vi "XML - Create XML file.vi"(8 "error in (no error)":errorcluster, 10 "Consolidated_CD":refnum<class "NIVS_Consolidated_CDW_MetaDataObj.lvclass">, 11 "CD Wizard - Internal Data":T1) -> (0 "error out":errorcluster)   [LabVIEW 2020, in "NIVS_Consolidated_CDW_MetaDataObj.lvclass"]
doc: "Create the XML file and alter the content of the file, so that it fits for the generated custom device."
uses:
  NIVS_Consolidated_CDW_MetaDataObj.lvclass
  Internal data.ctl
  C:/Program Files/National Instruments/LabVIEW 2024/resource/dialog/NewProjectWizard/MetaDataObj/MetaDataObj.lvclass
  Create XML-file - States.ctl
  <resource>/dialog/NewProjectWizard/MetaDataObj/MetaDataObj.lvclass/MetaDataObj.ctl
  NIVS_Consolidated_CDW_MetaDataObj.lvclass/NIVS_Consolidated_CDW_MetaDataObj.ctl
  Template Classes/NIVS_CD Template/NIVS_CD Template.lvclass/NIVS_CD Template.ctl
  CD System Explorer lvlib.ctl
  Target Type.ctl
  Template Classes/NIVS_CD Template/Read Submenu.vi
  Template Classes/NIVS_CD Template/Read Parent Menu.vi
  Template Classes/NIVS_CD Template/Read Max Instances.vi
  <resource>/dialog/NewProjectWizard/MetaDataObj/Accessors/Read Project Root.vi
  <resource>/dialog/NewProjectWizard/MetaDataObj/Accessors/Read Project Name.vi
  Read CD Template.vi
  CD System Explorer lvlib.vi
  Template Classes/NIVS_CD Template/NIVS_CD Template.lvclass
  <vilib>/Utility/Data Type/NI_Data Type.lvlib
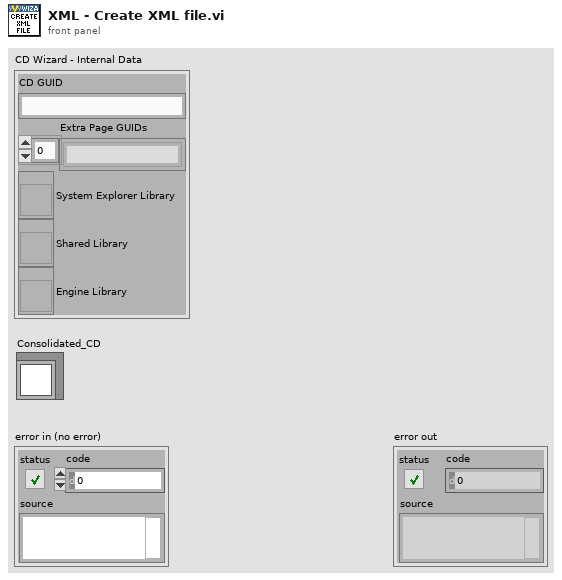
[diagram p1: front panel]
types:
  T1 = typedef "NIVS_Consolidated_CDW_MetaDataObj.lvclass/Internal data.ctl" = cluster{"CD GUID":string, "Extra Page GUIDs":string[], "System Explorer Library":refnum<vi>, "Shared Library":refnum<vi>, "Engine Library":refnum<vi>}
  T2 = typedef "NIVS_Consolidated_CDW_MetaDataObj.lvclass/Create XML-file - States.ctl" = enum16{"Read XML template file", "Change CD -MenuName-", "Change CD -Name-", "Change CD -Type-", "Change CD -Occurrences-", "Change CD -MainPageGUID-", "Change CD -InitVIPath-", "Change CD -WindowsCustomDeviceVIPath-", "Change CD -WindowsCustomDeviceVIRTPath-", "Change CD -Linuxx64CustomDeviceVIPath-", "Change CD -Linuxx64CustomDeviceVIRTPath-", "Change CD -MainPageVIPath-", "Change CD -ExtraPages-", "Change CD -ActionVIOnCompile-", "Change CD -ActionVIOnRecompile-", "Change CD -ExportConfigurationRTM-", "Write XML file content back"}
  T3 = typedef "NIVS_Consolidated_CDW_MetaDataObj.lvclass/CD System Explorer lvlib.ctl" = enum16{"LibraryFileName", "LibraryFolderName", "System Explorer.FolderName", "System Explorer.Dynamically Called.FolderName", "System Explorer.Dynamically Called.Extra Pages.FolderName", "System Explorer.Dynamically Called.Extra Pages.TemplatePathAndName", "System Explorer.Dynamically Called.Main Page.VIName", "System Explorer.Dynamically Called.Main Page.TemplatePathAndName", "System Explorer.Dynamically Called.Initialization VI.VIName", "System Explorer.Dynamically Called.Initialization VI.TemplatePathAndName", "System Explorer.SubVI.FolderName", "System Explorer.Types.FolderName", "System Explorer.ActionVIOnCompile.VIName", "System Explorer.ActionVIOnRecompile.VIName", "System Explorer.ExportConfigRTM.VIName", "System Explorer.PPL.ExportConfigRTM.VIName", "System Explorer.LoadHelpFile.VIName", "System Explorer.PPL.LoadHelpFile.VIName", "System Explorer.SetRTDriverVIsFilePaths.VIName", "System Explorer.ClearRTDriverVIs.VIName"}
  T4 = typedef "NIVS_Consolidated_CDW_MetaDataObj.lvclass/Target Type.ctl" = enum16{"Windows", "Linux x64"}
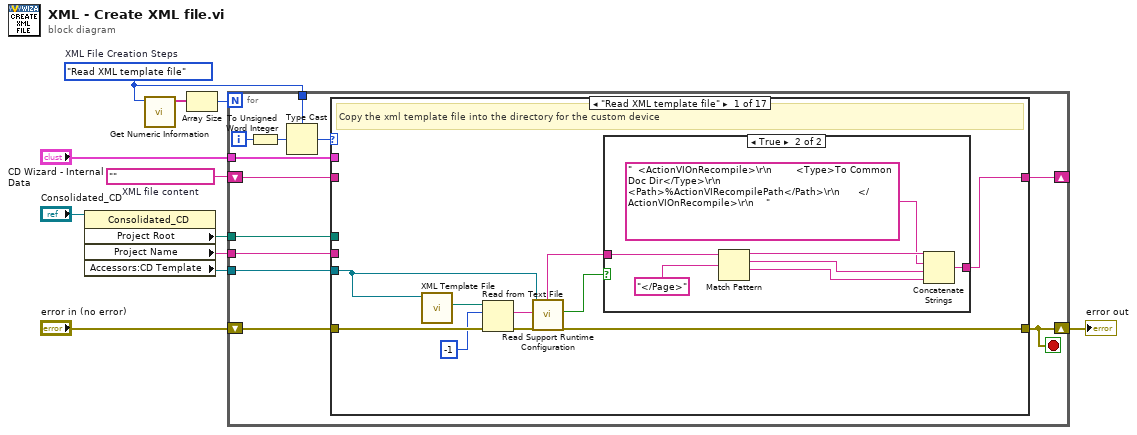
[diagram p0: block diagram]
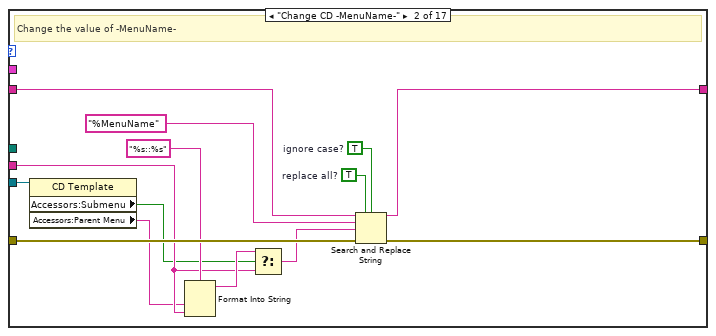
[diagram p3: hidden frame]
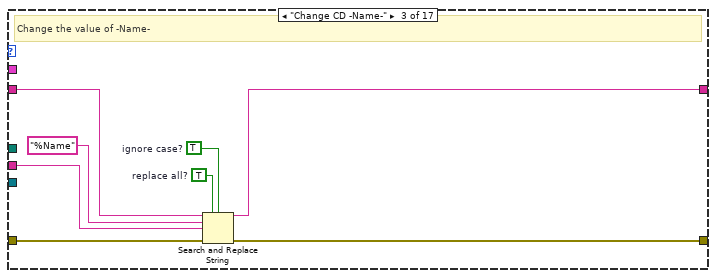
[diagram p4: hidden frame]
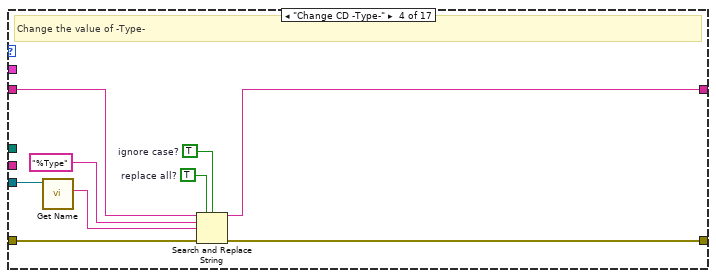
[diagram p5: hidden frame]
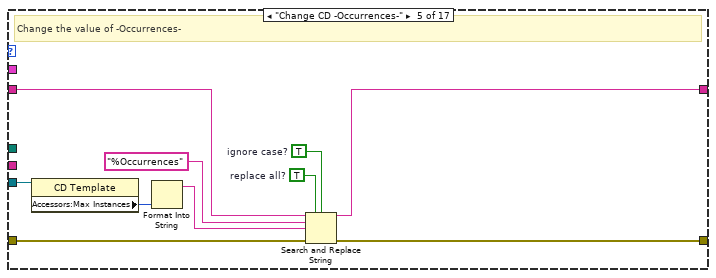
[diagram p6: hidden frame]
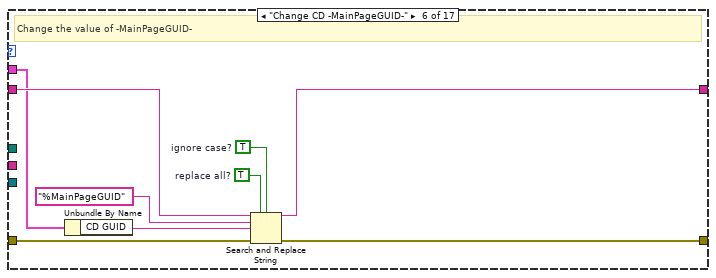
[diagram p7: hidden frame]
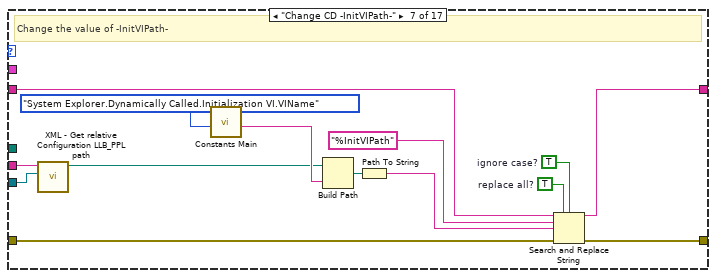
[diagram p8: hidden frame]
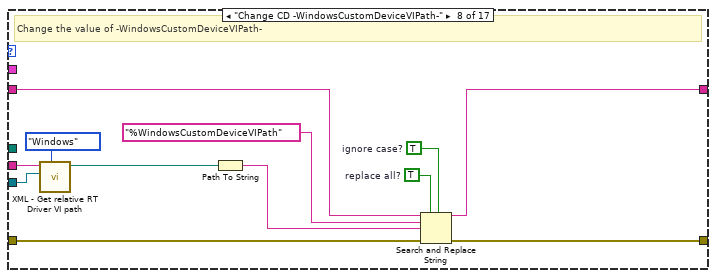
[diagram p9: hidden frame]
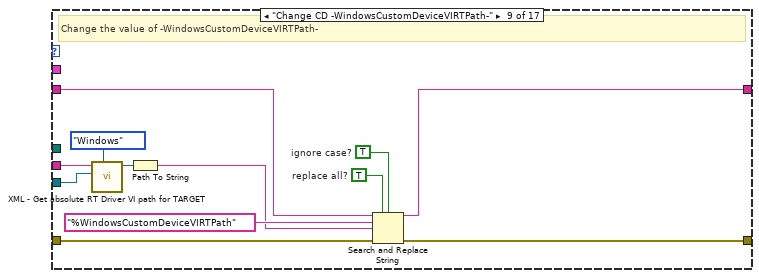
[diagram p10: hidden frame]
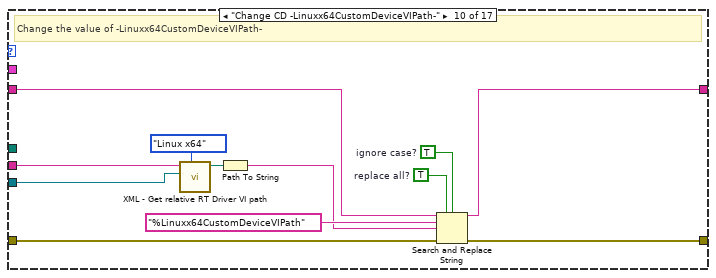
[diagram p11: hidden frame]
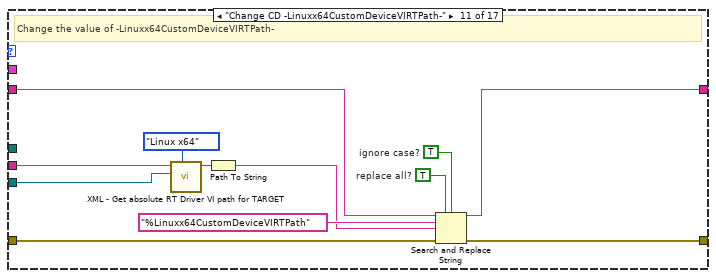
[diagram p12: hidden frame]
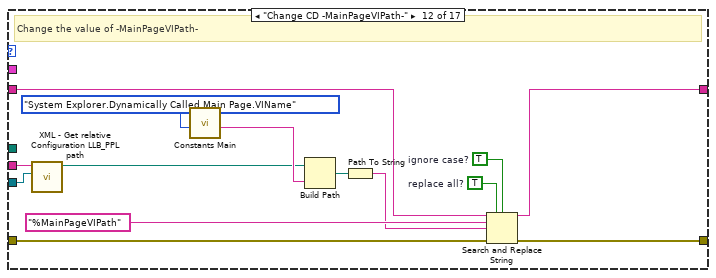
[diagram p13: hidden frame]
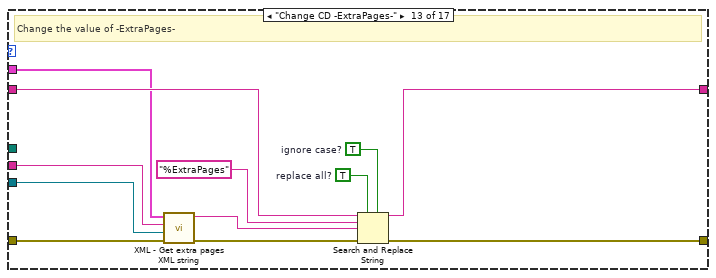
[diagram p14: hidden frame]
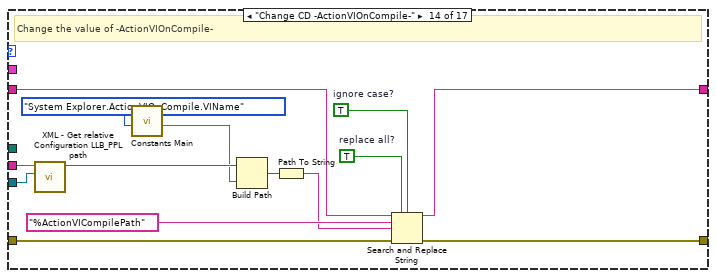
[diagram p15: hidden frame]
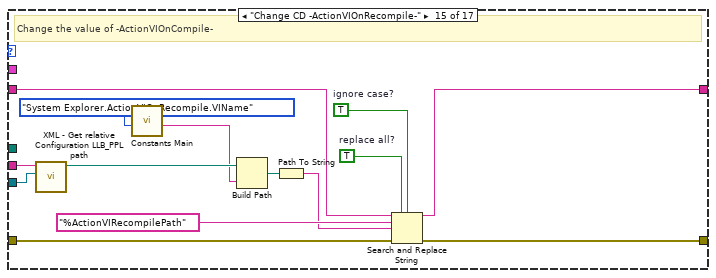
[diagram p16: hidden frame]
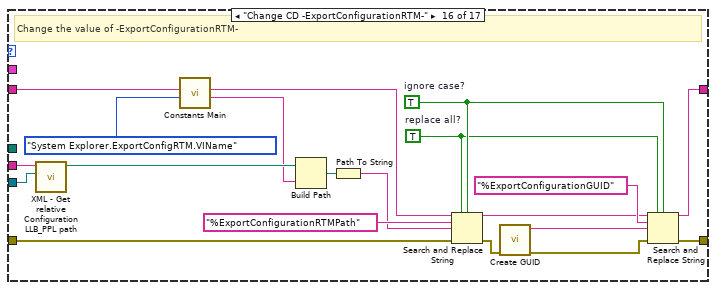
[diagram p17: hidden frame]
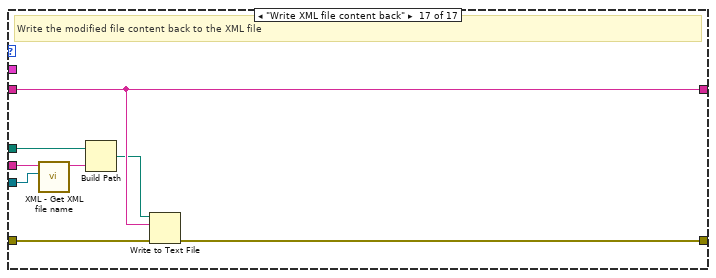
[diagram p18: hidden frame]
diagram:
  w2 = Create_XML-file_-_States."Read XML template file"  # XML File Creation Steps
  w10 = ""  # XML file content
  n1 = property class="Consolidated_CD"(reference="Consolidated_CD") -> ("Project Root"=w8:path, "Project Name"=w7:string, "Accessors:CD Template"=w6:refnum<class "NIVS_CD Template.lvclass">)  [unwired: 1 in, 2 out]
  n2 = call <vilib>:"Get Numeric Information.vi"("variant"=w2) -> ("enum names"=w3:string[])  [unwired: 7 in, 3 out]
  n3 = Array Size(array=w3) -> (size(s)=w4:i32)
  n4 = for {
    N: w4 -> [_]
    shift-right: [w18] -> w11
    shift-left: "error in (no error)" -> [w17]
    shift-right: [w22] -> _
    shift-left: w10 -> [w23]
    tunnel: w8 -> [w21]
    tunnel: w7 -> [w20]
    tunnel: w6 -> [w19]
    tunnel: w2 -> [w15]
    tunnel: "CD Wizard - Internal Data" -> [w12]
    i -> [w16]
    stop <- w18 stop-if-true
    # "While loop for State Machine"
    n5 = To Unsigned Word Integer(number=w16) -> (unsigned 16bit integer=w14:u16)
    n6 = Type Cast(type=w15, x=w14) -> (*(type *) &x=w13:T2)
    n7 = case shown="\"Read XML template file\"" w13 {
      tunnel: w17 -> [w32 w50 w58 w65 w72 w83 w93 w107 w119 w131 w143 w155 w169 w179 w193 w207 w230]
      tunnel: [w24 w51 w59 w68 w78 w87 w101 w115 w126 w138 w150 w163 w175 w189 w203 w210 w233] -> w18
      tunnel: w12 -> [_ _ _ _ _ w86 _ _ _ _ _ _ w173 _ _ _ _]
      tunnel: w23 -> [_ w53 w61 w70 w80 w89 w103 w112 w128 w140 w152 w165 w177 w191 w205 w224 w232]
      tunnel: [w28 w52 w60 w69 w79 w88 w102 w116 w127 w139 w151 w164 w176 w190 w204 w214 w232] -> w22
      tunnel: w21 -> [_ _ _ _ _ _ _ _ _ _ _ _ _ _ _ _ w229]
      tunnel: w20 -> [_ w44 w55 _ _ _ w92 w106 w118 w130 w142 w154 w168 w181 w195 w209 w228]
      tunnel: w19 -> [w27 w43 _ w64 w74 _ w91 w105 w117 w129 w141 w153 w167 w180 w194 w208 w227]
      frame "Read XML template file" {
        # "Copy the xml template file into the directory for the custom device"
        n8 = call-dynamic "XML Template File.vi"("CD Template"=w27) -> ("XML Template File"=w31:path)  [unwired: 10 in]
        n9 = Read from Text File(file (use dialog)=w31, count=-1, error in=w32) -> (text=w29:string, error out=w26:errorcluster)  [unwired: 1 in, 2 out]
        n10 = call "Read Support Runtime Configuration.vi"("error in"=w26, "NIVS_CD Template in"=w27) -> ("error out"=w24:errorcluster, "Support Runtime Configuration"=w25:bool)  [unwired: 7 in, 1 out]
        n11 = case shown="True" w25 {
          tunnel: w29 -> [w33 w37]
          tunnel: [w33 w36] -> w28
          frame False {
          }
          frame True {
            n12 = Match Pattern(string=w37, regular expression="</Page>" ("string")) -> (before substring=w40:string, match substring=w39:string, after substring=w34:string)  [unwired: 1 in, 1 out]
            n13 = Concatenate Strings(w40, "  <ActionVIOnRecompile>\r\n        <Type>To Common Doc Dir</Type>\r\n        <Path>%ActionVIRecompilePath</Path>\r\n      </ActionVIOnRecompile>\r\n    ", w39, w34) -> (w36:string)
          }
        }
      }
      frame "Change CD -MenuName-" {
        w48 = TRUE  # ignore case?
        w49 = TRUE  # replace all?
        # "Change the value of -MenuName-"
        n14 = property class="CD Template"(reference=w43) -> ("Accessors:Submenu"=w42:bool, "Accessors:Parent Menu"=w41:string)  [unwired: 1 in, 2 out]
        n15 = Format Into String(format string="%s::%s", w41, w44) -> (resulting string=w46:string)  [unwired: 2 in, 1 out]
        n16 = Select(t=w46, s=w42, f=w44) -> (s? t:f=w45:string)
        n17 = Search and Replace String(replace all?=w49, case sensitive?=w48, input string=w53, search string="%MenuName", replace string=w45, error in=w50) -> (result string=w52:string, error out=w51:errorcluster)  [unwired: 1 in, 3 out]
      }
      frame "Change CD -Name-" {
        w56 = TRUE  # ignore case?
        w57 = TRUE  # replace all?
        # "Change the value of -Name-"
        n18 = Search and Replace String(replace all?=w57, case sensitive?=w56, input string=w61, search string="%Name", replace string=w55, error in=w58) -> (result string=w60:string, error out=w59:errorcluster)  [unwired: 1 in, 3 out]
      }
      frame "Change CD -Type-" {
        w66 = TRUE  # ignore case?
        w67 = TRUE  # replace all?
        # "Change the value of -Type-"
        n19 = call-dynamic "Get Name.vi"("CD Template"=w64) -> ("String"=w63:string)  [unwired: 10 in]
        n20 = Search and Replace String(replace all?=w67, case sensitive?=w66, input string=w70, search string="%Type", replace string=w63, error in=w65) -> (result string=w69:string, error out=w68:errorcluster)  [unwired: 1 in, 3 out]
      }
      frame "Change CD -Occurrences-" {
        w75 = TRUE  # ignore case?
        w77 = TRUE  # replace all?
        # "Change the value of -Occurrences-"
        n21 = property class="CD Template"(reference=w74) -> ("Accessors:Max Instances"=w73:i32)  [unwired: 1 in, 2 out]
        n22 = Format Into String(w73) -> (resulting string=w76:string)  [unwired: 3 in, 1 out]
        n23 = Search and Replace String(replace all?=w77, case sensitive?=w75, input string=w80, search string="%Occurrences", replace string=w76, error in=w72) -> (result string=w79:string, error out=w78:errorcluster)  [unwired: 1 in, 3 out]
      }
      frame "Change CD -MainPageGUID-" {
        w82 = TRUE  # ignore case?
        w85 = TRUE  # replace all?
        # "Change the value of -MainPageGUID-"
        n24 = Unbundle By Name(w86) -> ("CD GUID"=w84:string)
        n25 = Search and Replace String(replace all?=w85, case sensitive?=w82, input string=w89, search string="%MainPageGUID", replace string=w84, error in=w83) -> (result string=w88:string, error out=w87:errorcluster)  [unwired: 1 in, 3 out]
      }
      frame "Change CD -InitVIPath-" {
        w99 = TRUE  # ignore case?
        w100 = TRUE  # replace all?
        # "Change the value of -InitVIPath-"
        n26 = call "XML - Get relative Configuration LLB_PPL path.vi"("CD Template"=w91, "Project Name"=w92) -> ("Relative Configuration LLB/PPL path"=w94:path)  [unwired: 9 in]
        n27 = call-poly "Constants Main.vi"("Action"=CD_System_Explorer_lvlib."System Explorer.Dynamically Called.Initialization VI.VIName") -> ("Output"=w97:string)  [unwired: 10 in]
        n28 = Build Path(base path=w94, name or relative path=w97) -> (appended path=w95:path)
        n29 = Path To String(path=w95) -> (string=w98:string)
        n30 = Search and Replace String(replace all?=w100, case sensitive?=w99, input string=w103, search string="%InitVIPath", replace string=w98, error in=w93) -> (result string=w102:string, error out=w101:errorcluster)  [unwired: 1 in, 3 out]
      }
      frame "Change CD -WindowsCustomDeviceVIPath-" {
        w113 = TRUE  # ignore case?
        w114 = TRUE  # replace all?
        # "Change the value of -WindowsCustomDeviceVIPath-"
        n31 = call "XML - Get relative RT Driver VI path.vi"("Target Type (Windows)"=Target_Type."Windows", "CD Template"=w105, "Project Name"=w106) -> ("Relative RT Driver VI path"=w108:path)  [unwired: 8 in]
        n32 = Path To String(path=w108) -> (string=w110:string)
        n33 = Search and Replace String(replace all?=w114, case sensitive?=w113, input string=w112, search string="%WindowsCustomDeviceVIPath", replace string=w110, error in=w107) -> (result string=w116:string, error out=w115:errorcluster)  [unwired: 1 in, 3 out]
      }
      frame "Change CD -WindowsCustomDeviceVIRTPath-" {
        w124 = TRUE  # ignore case?
        w125 = TRUE  # replace all?
        # "Change the value of -WindowsCustomDeviceVIRTPath-"
        n34 = call "XML - Get absolute RT Driver VI path for TARGET.vi"("Target Type (Windows)"=Target_Type."Windows", "CD Template"=w117, "Project Name"=w118) -> ("Relative RT Driver TARGET path"=w120:path)  [unwired: 8 in]
        n35 = Path To String(path=w120) -> (string=w122:string)
        n36 = Search and Replace String(replace all?=w125, case sensitive?=w124, input string=w128, search string="%WindowsCustomDeviceVIRTPath", replace string=w122, error in=w119) -> (result string=w127:string, error out=w126:errorcluster)  [unwired: 1 in, 3 out]
      }
      frame "Change CD -Linuxx64CustomDeviceVIPath-" {
        w136 = TRUE  # ignore case?
        w137 = TRUE  # replace all?
        # "Change the value of -Linuxx64CustomDeviceVIPath-"
        n37 = call "XML - Get relative RT Driver VI path.vi"("Target Type (Windows)"=Target_Type."Linux x64", "CD Template"=w129, "Project Name"=w130) -> ("Relative RT Driver VI path"=w132:path)  [unwired: 8 in]
        n38 = Path To String(path=w132) -> (string=w134:string)
        n39 = Search and Replace String(replace all?=w137, case sensitive?=w136, input string=w140, search string="%Linuxx64CustomDeviceVIPath", replace string=w134, error in=w131) -> (result string=w139:string, error out=w138:errorcluster)  [unwired: 1 in, 3 out]
      }
      frame "Change CD -Linuxx64CustomDeviceVIRTPath-" {
        w148 = TRUE  # ignore case?
        w149 = TRUE  # replace all?
        # "Change the value of -Linuxx64CustomDeviceVIRTPath-"
        n40 = call "XML - Get absolute RT Driver VI path for TARGET.vi"("Target Type (Windows)"=Target_Type."Linux x64", "CD Template"=w141, "Project Name"=w142) -> ("Relative RT Driver TARGET path"=w144:path)  [unwired: 8 in]
        n41 = Path To String(path=w144) -> (string=w145:string)
        n42 = Search and Replace String(replace all?=w149, case sensitive?=w148, input string=w152, search string="%Linuxx64CustomDeviceVIRTPath", replace string=w145, error in=w143) -> (result string=w151:string, error out=w150:errorcluster)  [unwired: 1 in, 3 out]
      }
      frame "Change CD -MainPageVIPath-" {
        w161 = TRUE  # ignore case?
        w162 = TRUE  # replace all?
        # "Change the value of -MainPageVIPath-"
        n43 = call "XML - Get relative Configuration LLB_PPL path.vi"("CD Template"=w153, "Project Name"=w154) -> ("Relative Configuration LLB/PPL path"=w156:path)  [unwired: 9 in]
        n44 = call-poly "Constants Main.vi"("Action"=CD_System_Explorer_lvlib."System Explorer.Dynamically Called.Main Page.VIName") -> ("Output"=w160:string)  [unwired: 10 in]
        n45 = Build Path(base path=w156, name or relative path=w160) -> (appended path=w158:path)
        n46 = Path To String(path=w158) -> (string=w157:string)
        n47 = Search and Replace String(replace all?=w162, case sensitive?=w161, input string=w165, search string="%MainPageVIPath", replace string=w157, error in=w155) -> (result string=w164:string, error out=w163:errorcluster)  [unwired: 1 in, 3 out]
      }
      frame "Change CD -ExtraPages-" {
        w171 = TRUE  # ignore case?
        w174 = TRUE  # replace all?
        # "Change the value of -ExtraPages-"
        n48 = call "XML - Get extra pages XML string.vi"("error in (no error)"=w169, "CD Template"=w167, "Project Name"=w168, "CD Wizard - Internal Data"=w173) -> ("error out"=w170:errorcluster, "Extra Pages XML string"=w172:string)  [unwired: 6 in]
        n49 = Search and Replace String(replace all?=w174, case sensitive?=w171, input string=w177, search string="%ExtraPages", replace string=w172, error in=w170) -> (result string=w176:string, error out=w175:errorcluster)  [unwired: 1 in, 3 out]
      }
      frame "Change CD -ActionVIOnCompile-" {
        w187 = TRUE  # ignore case?
        w188 = TRUE  # replace all?
        # "Change the value of -ActionVIOnCompile-"
        n50 = call "XML - Get relative Configuration LLB_PPL path.vi"("CD Template"=w180, "Project Name"=w181) -> ("Relative Configuration LLB/PPL path"=w186:path)  [unwired: 9 in]
        n51 = call-poly "Constants Main.vi"("Action"=CD_System_Explorer_lvlib."System Explorer.ActionVIOnCompile.VIName") -> ("Output"=w182:string)  [unwired: 10 in]
        n52 = Build Path(base path=w186, name or relative path=w182) -> (appended path=w185:path)
        n53 = Path To String(path=w185) -> (string=w184:string)
        n54 = Search and Replace String(replace all?=w188, case sensitive?=w187, input string=w191, search string="%ActionVICompilePath", replace string=w184, error in=w179) -> (result string=w190:string, error out=w189:errorcluster)  [unwired: 1 in, 3 out]
      }
      frame "Change CD -ActionVIOnRecompile-" {
        w201 = TRUE  # ignore case?
        w202 = TRUE  # replace all?
        # "Change the value of -ActionVIOnCompile-"
        n55 = call "XML - Get relative Configuration LLB_PPL path.vi"("CD Template"=w194, "Project Name"=w195) -> ("Relative Configuration LLB/PPL path"=w200:path)  [unwired: 9 in]
        n56 = call-poly "Constants Main.vi"("Action"=CD_System_Explorer_lvlib."System Explorer.ActionVIOnRecompile.VIName") -> ("Output"=w196:string)  [unwired: 10 in]
        n57 = Build Path(base path=w200, name or relative path=w196) -> (appended path=w199:path)
        n58 = Path To String(path=w199) -> (string=w198:string)
        n59 = Search and Replace String(replace all?=w202, case sensitive?=w201, input string=w205, search string="%ActionVIRecompilePath", replace string=w198, error in=w193) -> (result string=w204:string, error out=w203:errorcluster)  [unwired: 1 in, 3 out]
      }
      frame "Change CD -ExportConfigurationRTM-" {
        w217 = TRUE  # ignore case?
        w216 = TRUE  # replace all?
        # "Change the value of -ExportConfigurationRTM-"
        n60 = call "XML - Get relative Configuration LLB_PPL path.vi"("CD Template"=w208, "Project Name"=w209) -> ("Relative Configuration LLB/PPL path"=w223:path)  [unwired: 9 in]
        n61 = call-poly "Constants Main.vi"("Action"=CD_System_Explorer_lvlib."System Explorer.ExportConfigRTM.VIName") -> ("Output"=w219:string)  [unwired: 10 in]
        n62 = Build Path(base path=w223, name or relative path=w219) -> (appended path=w222:path)
        n63 = Path To String(path=w222) -> (string=w221:string)
        n64 = Search and Replace String(replace all?=w216, case sensitive?=w217, input string=w224, search string="%ExportConfigurationRTMPath", replace string=w221, error in=w207) -> (result string=w215:string, error out=w213:errorcluster)  [unwired: 1 in, 3 out]
        n65 = call "Create GUID.vi"("error in (no error)"=w213) -> ("error out"=w211:errorcluster, "Generated GUID"=w212:string)  [unwired: 9 in]
        n66 = Search and Replace String(replace all?=w216, case sensitive?=w217, input string=w215, search string="%ExportConfigurationGUID", replace string=w212, error in=w211) -> (result string=w214:string, error out=w210:errorcluster)  [unwired: 1 in, 3 out]
      }
      frame "Write XML file content back" {
        # "Write the modified file content back to the XML file"
        n67 = call "XML - Get XML file name.vi"("CD Template"=w227, "CD Name"=w228) -> ("XML file name"=w231:string)  [unwired: 9 in]
        n68 = Build Path(base path=w229, name or relative path=w231) -> (appended path=w226:path)
        n69 = Write to Text File(file (use dialog)=w226, text=w232, error in=w230) -> (error out=w233:errorcluster)  [unwired: 3 out]
      }
    }
  }
  "error out" <- w11
